vi "pair modules.vi"(5 "Paired Target Configuration":refnum<class "PL_Target Configuration.lvclass">, 6 "paired engine in":refnum<class "engine configuration.lvclass">, 7 "Target Configuration":refnum<class "PL_Target Configuration.lvclass">, 8 "error in":errorcluster, 9 "engine configuration in":refnum<class "engine configuration.lvclass">, 10 "module to pair with":refnum<class "TEC editor node.lvclass">, 11 "UDP Broadcast Editor Node in":refnum<class "TEC editor node.lvclass">) -> (0 "error out":errorcluster, 1 "engine configuration out":refnum<class "engine configuration.lvclass">, 2 "module to pair with out":refnum<class "TEC editor node.lvclass">, 3 "UDP Broadcast Editor Node out":refnum<class "TEC editor node.lvclass">, 4 "paired engine out":refnum<class "engine configuration.lvclass">)   [LabVIEW 2014, in "TEC editor node.lvclass"]
uses:
  TEC editor node.lvclass
  <vilib>/NI/Module Execution Interface/Engine Configuration/engine configuration.lvclass
  <vilib>/NI/DCAF/Tag Editor Core/Framework Configuration Classes/target configuration/PL_Target Configuration.lvclass
  <vilib>/NI/DCAF/Tag Editor Core/Framework Configuration Classes/target configuration/PL_Target Configuration.lvclass/PL_Target Configuration.ctl
  TEC editor node.lvclass/TEC editor node.ctl
  <vilib>/NI/Configuration Framework/serializable configuration/NISE_CEF_serializable configuration.lvclass/NISE_CEF_serializable configuration.ctl
  configuration/TEC configuration.lvclass/TEC configuration.ctl
  configuration/Read send to port.vi
  configuration/Read receive on port.vi
  configuration/Write send to address.vi
  configuration/Write receive on port.vi
  configuration/Write send to port.vi
  <vilib>/NI/DCAF/Tag Editor Core/Framework Configuration Classes/target configuration/Read hostname.vi
  <vilib>/Utility/LVClass/Get LV Class Name.vi
  <vilib>/NI/Configuration Framework/error generator/NISE_error generator.vi
  configuration/TEC configuration.lvclass
  <vilib>/NI/Configuration Framework/serializable configuration/NISE_CEF_serializable configuration.lvclass
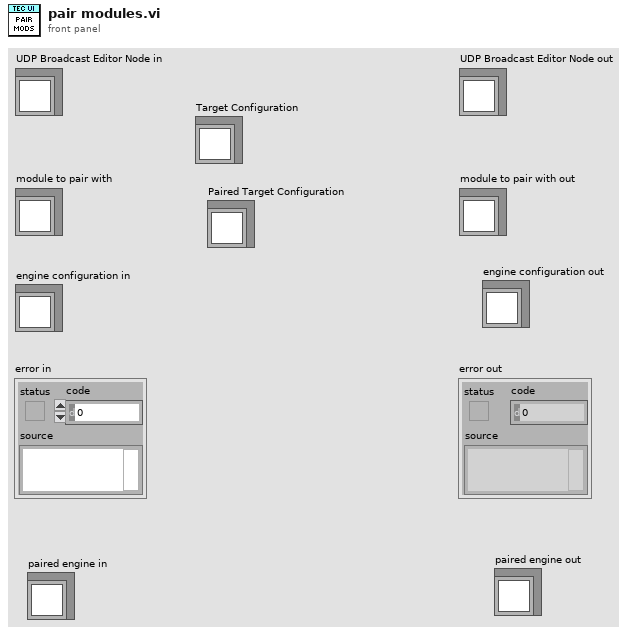
[diagram p1: front panel]
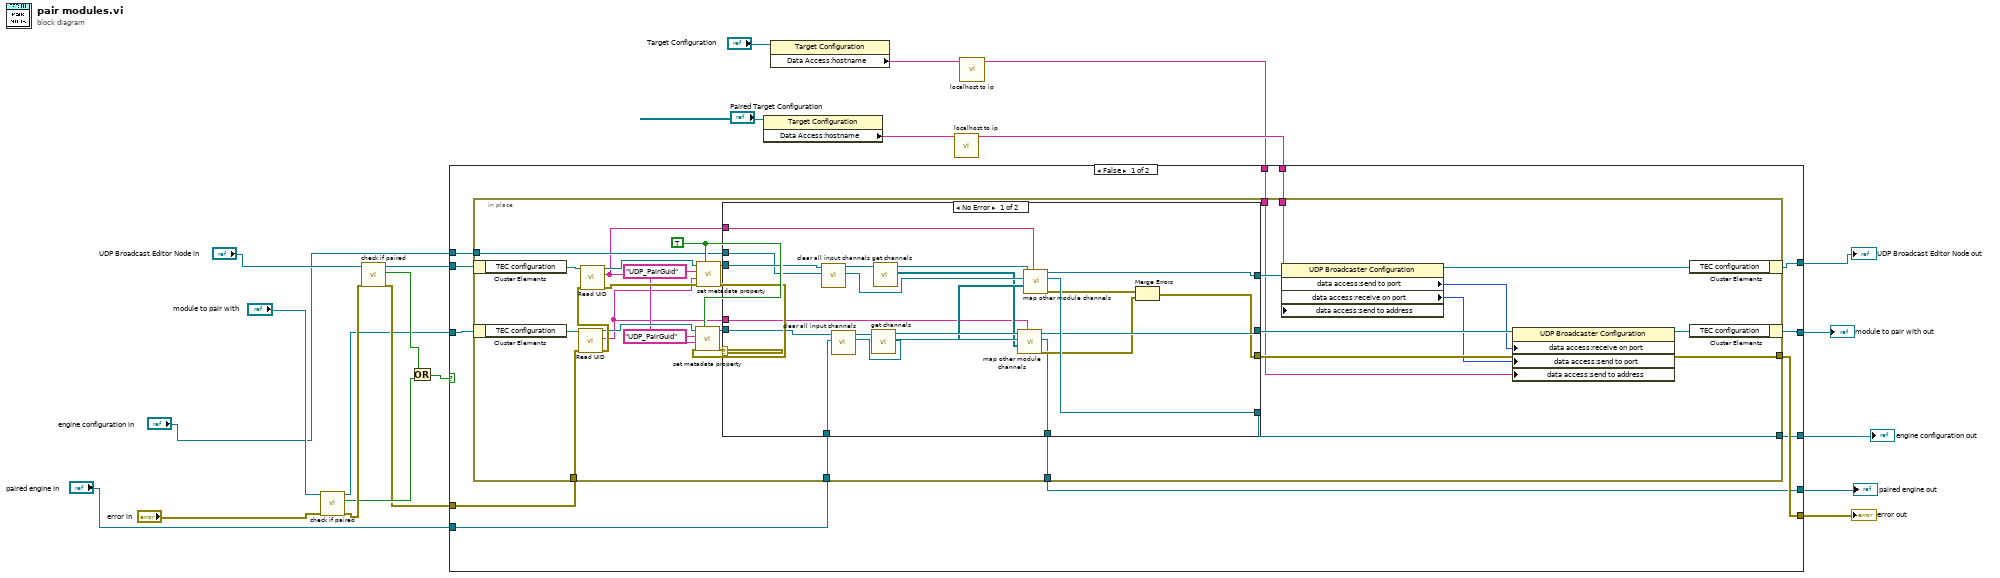
[diagram p0: block diagram]
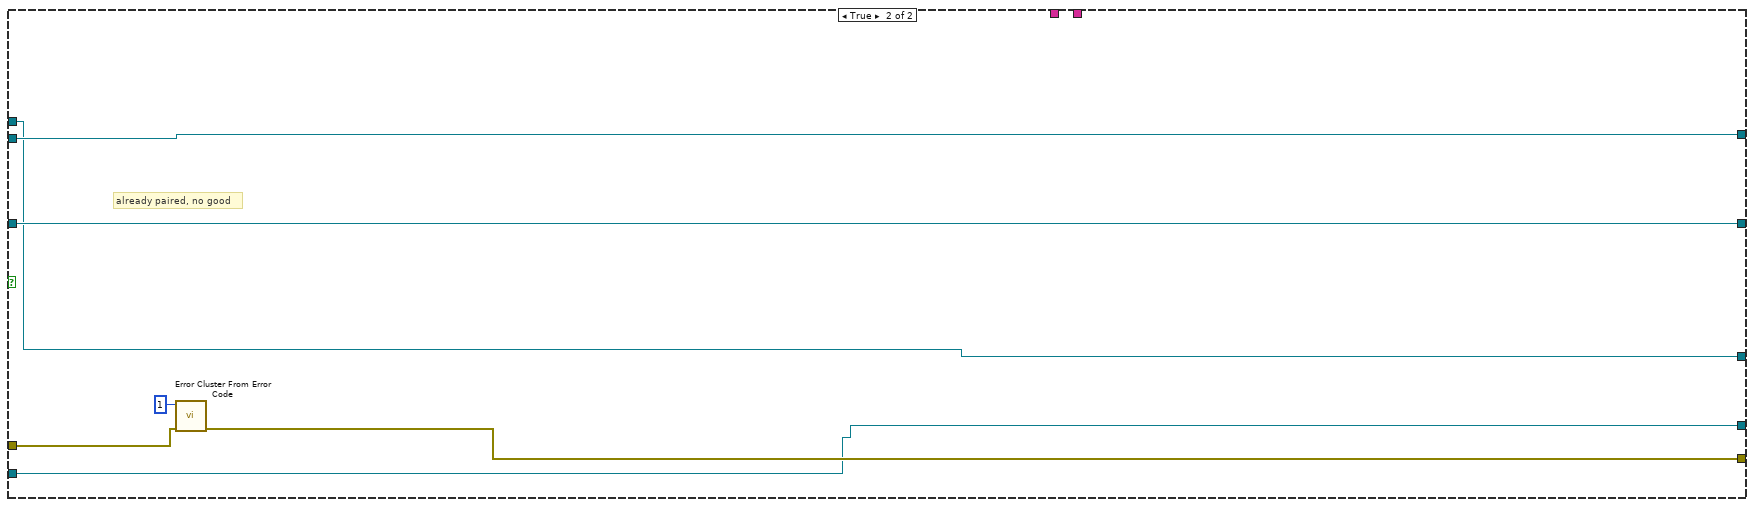
[diagram p3: hidden frame]
diagram:
  n1 = call "check if paired.vi"("error in"="error in", "UDP Broadcast Editor Node in"="module to pair with") -> ("error out"=w20:errorcluster, "paired"=w18:bool, "UDP Broadcast Editor Node out"=w12:refnum<class "TEC editor node.lvclass">)  [unwired: 7 in]
  n2 = call "check if paired.vi"("error in"=w20, "UDP Broadcast Editor Node in"="UDP Broadcast Editor Node in") -> ("error out"=w16:errorcluster, "paired"=w19:bool, "UDP Broadcast Editor Node out"=w13:refnum<class "TEC editor node.lvclass">)  [unwired: 7 in]
  n3 = Or(x=w19, y=w18) -> (x .or. y?=w17:bool)
  n4 = property class="Target Configuration"(reference="Paired Target Configuration") -> ("Data Access:hostname"=w4:string)  [unwired: 1 in, 2 out]
  n5 = property class="Target Configuration"(reference="Target Configuration") -> ("Data Access:hostname"=w2:string)  [unwired: 1 in, 2 out]
  n6 = call "localhost to ip.vi"("hostname"=w4) -> ("true hostname"=w3:string)  [unwired: 10 in]
  n7 = call "localhost to ip.vi"("hostname"=w2) -> ("true hostname"=w1:string)  [unwired: 10 in]
  n8 = case shown="False" w17 {
    tunnel: w16 -> [w32 w97]
    tunnel: [w31 w95] -> w15
    tunnel: [w34 w94] -> w14
    tunnel: w13 -> [w35 w94]
    tunnel: w12 -> [w33 w93]
    tunnel: [w30 w93] -> w11
    tunnel: "engine configuration in" -> [w29 w92]
    tunnel: "paired engine in" -> [w28 w91]
    tunnel: [w27 w92] -> w8
    tunnel: [w26 w91] -> w7
    tunnel: w1 -> [w25 _]
    tunnel: w3 -> [w24 _]
    frame False {
      n9 = in-place {
        in-place-border: w32 -> [w62]
        in-place-border: [w52] -> w31
        in-place-border: w29 -> [w47]
        in-place-border: w28 -> [w46]
        in-place-border: [w44] -> w27
        in-place-border: [w43] -> w26
        in-place-border: w25 -> [w37]
        in-place-border: w24 -> [w36]
        w58 = TRUE ("overwrite?")
        n10 = in-place-cluster #1(w35) -> ("TEC configuration"=w64:refnum<class "TEC configuration.lvclass">)
        n11 = in-place-cluster #2(w33) -> ("TEC configuration"=w63:refnum<class "TEC configuration.lvclass">)
        n12 = call <vilib>:"Read UID.vi"("error in"=w62, "configuration in"=w63) -> ("error out"=w61:errorcluster, "instance id"=w42:string, "configuration out"=w56:refnum<class "TEC configuration.lvclass">)  [unwired: 7 in]
        n13 = call <vilib>:"Read UID.vi"("error in"=w61, "configuration in"=w64) -> ("error out"=w55:errorcluster, "instance id"=w45:string, "configuration out"=w57:refnum<class "TEC configuration.lvclass">)  [unwired: 7 in]
        n14 = call <vilib>:"set metadata property.vi"("overwrite?"=w58, "error in"=w55, "value"=w42, "key"="UDP_PairGuid", "configuration in"=w57) -> ("error out"=w54:errorcluster, "configuration out"=w48:refnum<class "TEC configuration.lvclass">)  [unwired: 5 in]
        n15 = call <vilib>:"set metadata property.vi"("overwrite?"=w58, "error in"=w54, "value"=w45, "key"="UDP_PairGuid", "configuration in"=w56) -> ("error out"=w53:errorcluster, "configuration out"=w51:refnum<class "TEC configuration.lvclass">)  [unwired: 5 in]
        n16 = case shown="No Error" w53 {
          selector: w53 -> [_ w90]
          tunnel: [w71 w90] -> w52
          tunnel: w51 -> [w85 w89]
          tunnel: [w72 w89] -> w50
          tunnel: [w77 w88] -> w49
          tunnel: w48 -> [w84 w88]
          tunnel: w47 -> [w81 w86]
          tunnel: w46 -> [w79 w87]
          tunnel: w45 -> [w74 _]
          tunnel: [w76 w86] -> w44
          tunnel: [w69 w87] -> w43
          tunnel: w42 -> [w65 _]
          frame No Error {
            n17 = call "clear all input channels.vi"("engine configuration in"=w81, "TEC configuration in"=w84) -> ("engine configuration out"=w80:refnum<class "engine configuration.lvclass">, "TEC configuration out"=w83:refnum<class "TEC configuration.lvclass">)  [unwired: 8 in]
            n18 = call "clear all input channels.vi"("engine configuration in"=w79, "TEC configuration in"=w85) -> ("engine configuration out"=w68:refnum<class "engine configuration.lvclass">, "TEC configuration out"=w82:refnum<class "TEC configuration.lvclass">)  [unwired: 8 in]
            n19 = call-dynamic "get channels.vi"("TEC configuration in"=w82) -> ("channels"=w67:refnum<class "TBM channel.lvclass">[], "TEC configuration out"=w73:refnum<class "TEC configuration.lvclass">)  [unwired: 9 in]
            n20 = call-dynamic "get channels.vi"("TEC configuration in"=w83) -> ("channels"=w66:refnum<class "TBM channel.lvclass">[], "TEC configuration out"=w78:refnum<class "TEC configuration.lvclass">)  [unwired: 9 in]
            n21 = call "map other module channels.vi"("instance id"=w65, "channels"=w66, "engine configuration in"=w68, "TEC configuration in"=w73) -> ("error out"=w70:errorcluster, "engine configuration out"=w69:refnum<class "engine configuration.lvclass">, "TEC configuration out"=w72:refnum<class "TEC configuration.lvclass">)  [unwired: 5 in]
            n22 = call "map other module channels.vi"("instance id"=w74, "channels"=w67, "engine configuration in"=w80, "TEC configuration in"=w78) -> ("error out"=w75:errorcluster, "engine configuration out"=w76:refnum<class "engine configuration.lvclass">, "TEC configuration out"=w77:refnum<class "TEC configuration.lvclass">)  [unwired: 5 in]
            n23 = Merge Errors(w75, w70) -> (w71:errorcluster)
          }
          frame Error {
          }
        }
        n24 = property class="UDP Broadcaster Configuration"(reference=w49, "data access:send to address"=w36) -> (reference out=w40:refnum<class "TEC configuration.lvclass">, "data access:send to port"=w38:u16, "data access:receive on port"=w39:u16)  [unwired: 1 in, 1 out]
        n25 = property class="UDP Broadcaster Configuration"(reference=w50, "data access:receive on port"=w38, "data access:send to port"=w39, "data access:send to address"=w37) -> (reference out=w41:refnum<class "TEC configuration.lvclass">)  [unwired: 1 in, 1 out]
        n26 = in-place-cluster #1("TEC configuration"=w40) -> (w34:refnum<class "TEC editor node.lvclass">)
        n27 = in-place-cluster #2("TEC configuration"=w41) -> (w30:refnum<class "TEC editor node.lvclass">)
      }
    }
    frame True {
      # "already paired, no good"
      n28 = call <vilib>:"Error Cluster From Error Code.vi"("error in (no error)"=w97, "error code (0)"=1) -> ("error out"=w95:errorcluster)  [unwired: 7 in]
    }
  }
  "error out" <- w15
  "UDP Broadcast Editor Node out" <- w14
  "module to pair with out" <- w11
  "engine configuration out" <- w8
  "paired engine out" <- w7
